vi "query NR HO Operation Band.vi"(8 "error in (no error)":errorcluster caption="에러 입력(에러 없음)", 10 "Selected CC Argements":T1, 11 "Anritsu Call Box_Implement 입력":refnum<class "Anritsu Call Box_Implement.lvclass">) -> (0 "error out":errorcluster caption="에러 출력", 2 "Operation Band":u32, 3 "Anritsu Call Box_Implement 출력":refnum<class "Anritsu Call Box_Implement.lvclass">)   [LabVIEW 2023, in "ANRITSU Call Box.lvlib" / "Anritsu Call Box_Implement.lvclass"]
uses:
  Anritsu Call Box_Implement.lvclass
  Anritsu Call Box_Implement.lvclass/Anritsu Call Box_Implement.ctl
  NR/NR.lvclass
  Type Definition/NR Selected CC Type Arguments.ctl
  ANRITSU Call Box.lvlib
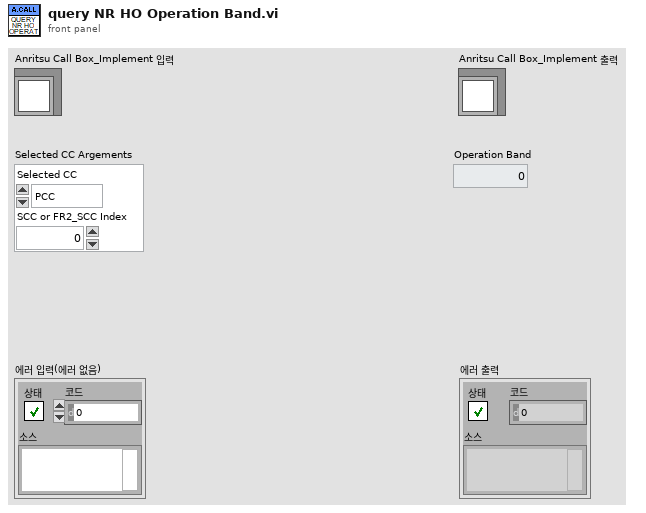
[diagram p1: front panel]
types:
  T1 = typedef "ANRITSU Call Box.lvlib/NR Selected CC Type Arguments.ctl" = cluster{"Selected CC":enum16{"PCC", "SCC", "FR2_PCC", "FR2_SCC"}, "SCC or FR2_SCC Index":u32}
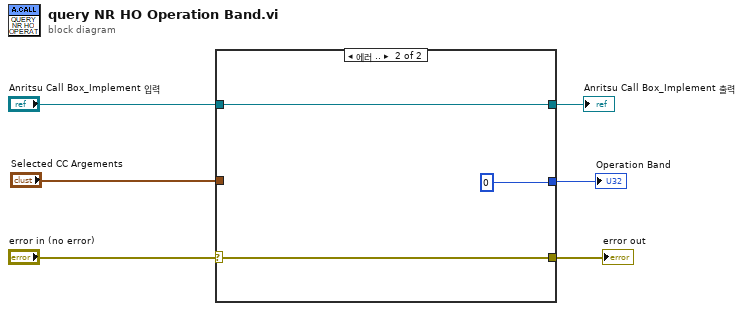
[diagram p0: block diagram]
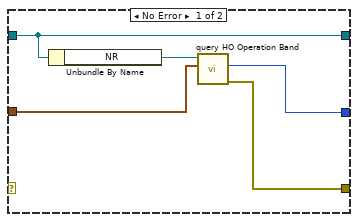
[diagram p2: hidden frame]
diagram:
  n1 = case shown="에러 .." "error in (no error)" {
    selector: "error in (no error)" -> [_ w13]
    tunnel: "Anritsu Call Box_Implement 입력" -> [w11 w14]
    tunnel: [w11 w14] -> w2
    tunnel: [w7 w13] -> w1
    tunnel: "Selected CC Argements" -> [w9 _]
    tunnel: [w8 u32 0 ("Operation Band")] -> w3
    frame No Error {
      n2 = Unbundle By Name(w11) -> ("NR"=w10:refnum<class "NR.lvclass">)
      n3 = call "query HO Operation Band.vi"("Selected CC Argements"=w9, "NR 입력"=w10) -> ("error out"=w7:errorcluster, "Operation Band"=w8:u32)  [unwired: 7 in, 1 out]
    }
    frame Error {
    }
  }
  "error out" <- w1
  "Anritsu Call Box_Implement 출력" <- w2
  "Operation Band" <- w3
